vi "test_ThreeSessThreePinTwoInstrTwoSiteReservation_CallGetConnectionsFromPinForAllDcPowerPinsAllSites_ReturnsThreeConnections.vi"(8 "error in":errorcluster) -> (0 "error out":errorcluster, 2 "result":string, 3 "pass":bool)   [LabVIEW 2021, in "MeasurementServerTests.lvlib"]
uses:
  MeasurementServerTests.lvlib
  Runtime/Clients/Session Management V1/Session Reservation/Connection with Session.ctl
  Runtime/Clients/Session Management V1/Session Reservation/Connection.ctl
  Runtime/Sessions/niDCPower/Session Factory/Session Factory.lvclass
  C:/dev/measurementlink-labview/Source/Runtime/Sessions/Instrument/ISession Factory/ISession Factory.lvclass
  Runtime/Clients/Session Management V1/Session Reservation/Pin Type.ctl
  e462a96d-9dce-4a61-b4bd-fba70dd973b3.vi
  da43ad04-91ae-4dbc-8eb3-60d6b08c7e97.vi
  481e2142-dde9-4265-ba9c-fc6a4d123327.vi
  514a39f3-05c6-4c8c-919b-303d9a210aef.vi
  c8103fad-7484-438a-bb86-fb7f0b67a6c2.vi
  514a39f3-05c6-4c8c-919b-303d9a210aef.vi/10aac40e-32b1-41e4-9263-c4508fa95940.vi
  Runtime/Clients/Session Management V1/Session Reservation/Pin to Pin Array.vi
  <vilib>/AdvancedString/1D String Array to Delimited String.vi
  c8103fad-7484-438a-bb86-fb7f0b67a6c2.vi/94283ac5-2298-4b3a-b57d-7be67da3787d.vi
  c8103fad-7484-438a-bb86-fb7f0b67a6c2.vi/f7d9c9cb-0251-4d67-81cb-70e1b0e8b69f.vi
  c8103fad-7484-438a-bb86-fb7f0b67a6c2.vi/48d9c053-c3ce-4ae4-8653-846fcb37df32.vi
  c8103fad-7484-438a-bb86-fb7f0b67a6c2.vi/38a8d12d-9165-42a0-bd04-ad62bed472d1.vi
  Runtime/Clients/Session Management V1/Session Reservation/Get Connections Impl.vi
  <vilib>/JDP Science/JSONtext/Variant to JSON Text.vi
  <vilib>/JDP Science/JSONtext/LVClass Serializer/JSONtext LVClass Serializer.lvclass
  Runtime/Clients/Session Management V1/Session Reservation/Session Reservation.lvclass
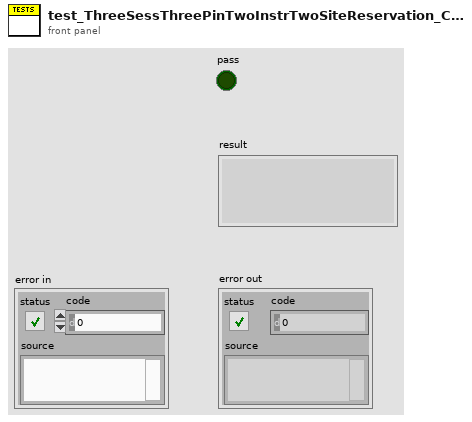
[diagram p1: front panel]
types:
  T1 = typedef "NI Session Management V1 Client.lvlib/Session Reservation.lvclass/Pin Type.ctl" = enum16{"DUT and System Pins", "System Pins"}
  T2 = typedef "NI Session Management V1 Client.lvlib/Session Reservation.lvclass/Connection.ctl" = cluster{"pin or relay name":string, "site":i32, "instrument type id":string, "channel":string}
  T3 = typedef "NI Session Management V1 Client.lvlib/Session Reservation.lvclass/Connection with Session.ctl" = cluster{"connection":T2, "session":variant}
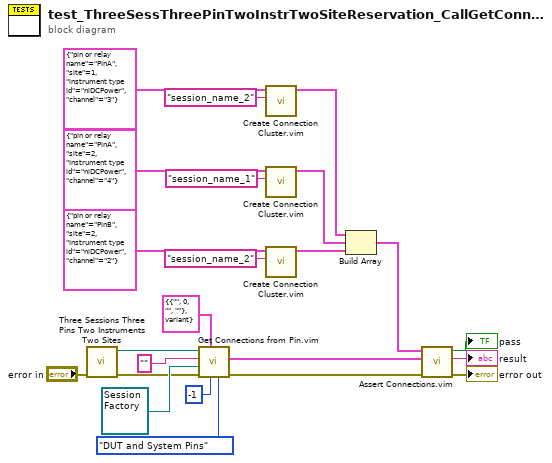
[diagram p0: block diagram]
diagram:
  n1 = call "Three Sessions Three Pins Two Instruments Two Sites.vi"("error in"="error in") -> ("error out"=w4:errorcluster, "session reservation out"=w3:refnum<class "Session Reservation.lvclass">)  [unwired: 8 in, 1 out]
  n2 = call "Get Connections from Pin.vim"("pin type"=Pin_Type."DUT and System Pins", "site"=-1, "connection type"=T3 {"connection"={"pin or relay name"="", "site"=0, "instrument type id"="", "channel"=""}, "session"=variant} ("connection"), "error in"=w4, "session factory"=refnum<class "Session Factory.lvclass"> refnum ("MeasurementLink niDCPower.lvlib:Instrument.lvclass"), "pin or relay name"="", "session reservation in"=w3) -> ("error out"=w2:errorcluster, "connections"=w23:T3[])  [unwired: 2 in, 1 out]
  n3 = call "Create Connection Cluster.vim"("session in"="session_name_2", "hardware independent connection in"=T2 {"pin or relay name"="PinA", "site"=1, "instrument type id"="niDCPower", "channel"="3"} ("connection")) -> ("connection out"=w20:T3)  [unwired: 9 in]
  n4 = call "Create Connection Cluster.vim"("session in"="session_name_1", "hardware independent connection in"=T2 {"pin or relay name"="PinA", "site"=2, "instrument type id"="niDCPower", "channel"="4"} ("connection")) -> ("connection out"=w11:T3)  [unwired: 9 in]
  n5 = call "Create Connection Cluster.vim"("session in"="session_name_2", "hardware independent connection in"=T2 {"pin or relay name"="PinB", "site"=2, "instrument type id"="niDCPower", "channel"="2"} ("connection")) -> ("connection out"=w7:T3)  [unwired: 9 in]
  n6 = Build Array(w20, w11, w7) -> (w19:T3[])
  n7 = call "Assert Connections.vim"("error in"=w2, "actual connections"=w23, "expected connections"=w19) -> ("error out"=→"error out":errorcluster, "result"=→"result":string, "pass"=→"pass":bool)  [unwired: 6 in]
